vi "Write to AO Channel.vi"(8 "error in":errorcluster, 10 "ctrlMotorControl":dbl, 11 "DAQ Device":T2) -> (0 "error out":errorcluster, 2 "ctrlMotorControl written":dbl, 3 "Analog Output Cluster":T1)   [LabVIEW 2021]
uses:
  DAQNav Cluster.ctl
  Analog Cluster.ctl
  <userlib>/DAQNavi Polymorphic VI/write/DAQNavi Write (Analog DBL 1Chan 1Samp).vi
panel:
  in  "Parameter Name":string
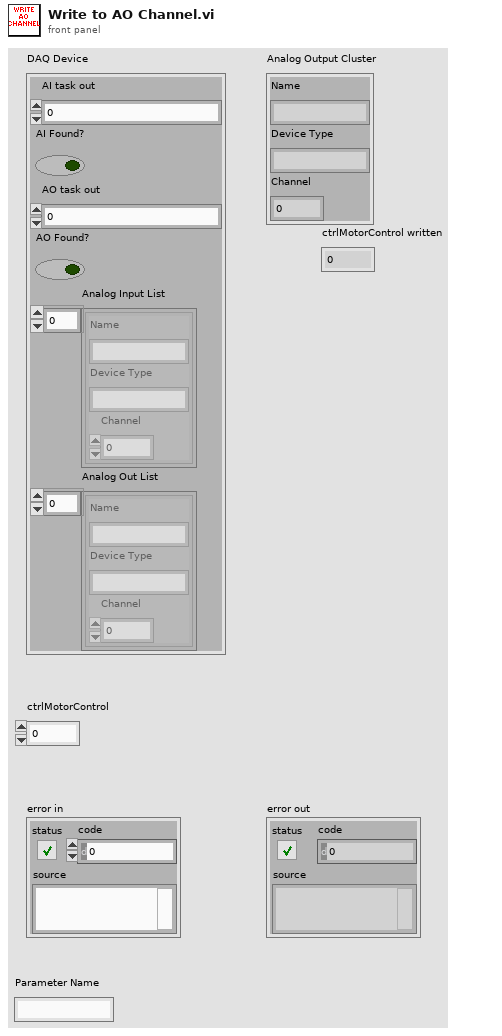
[diagram p1: front panel]
types:
  T1 = typedef "Analog Cluster.ctl" = cluster{"Name":string, "Device Type":string, "Channel":i32}
  T2 = typedef "DAQNav Cluster.ctl" = cluster{"AI task out":i32, "AI Found?":bool, "AO task out":i32, "AO Found?":bool, "Analog Input List":T1[], "Analog Out List":T1[]}
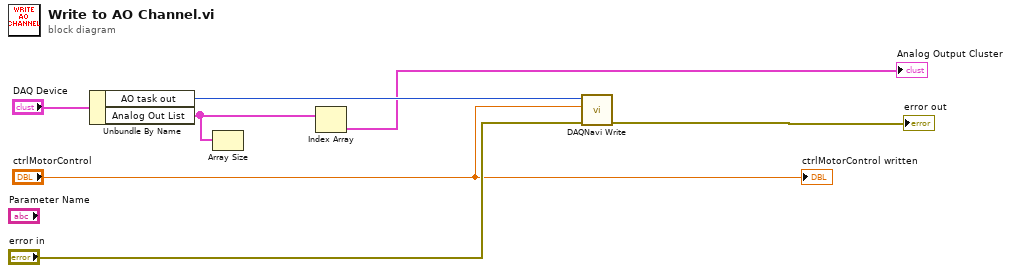
[diagram p0: block diagram]
diagram:
  n1 = Unbundle By Name("DAQ Device") -> ("AO task out"=w5:i32, "Analog Out List"=w3:T1[])
  n2 = Array Size(array=w3) -> ()  [unwired: 1 out]
  n3 = Index Array(array=w3) -> (element=→"Analog Output Cluster":T1)  [unwired: 1 in]
  n4 = call-poly <userlib>:"DAQNavi Write.vi"("error in (no error)"="error in", "data"="ctrlMotorControl", "task in"=w5) -> ("error out"=→"error out":errorcluster)  [unwired: 6 in, 2 out]
  "ctrlMotorControl written" <- "ctrlMotorControl"
